vi "rename tag.vi"(7 "owner ID":string, 8 "error in":errorcluster, 9 "new name":string, 10 "old name":string, 11 "engine configuration in":refnum<class "engine configuration.lvclass">) -> (0 "error out":errorcluster, 3 "engine configuration out":refnum<class "engine configuration.lvclass">)   [LabVIEW 2014, in "engine configuration.lvclass"]
doc: "This function is used to rename a tag. If a tag claims to have an owner, only that owner is allowed to modify the tag name."
uses:
  engine configuration.lvclass
  <vilib>/NI/Tag Bus/tag/tag descriptor.lvclass
  <vilib>/NI/Tag Bus/tag/tag descriptor.lvclass/tag descriptor.ctl
  engine configuration.lvclass/engine configuration.ctl
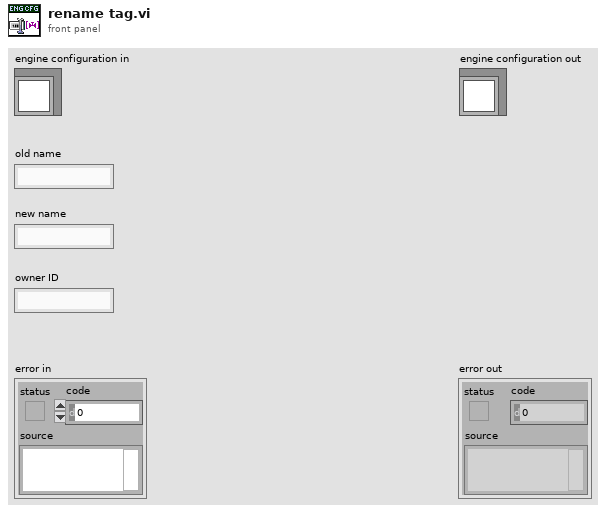
[diagram p1: front panel]
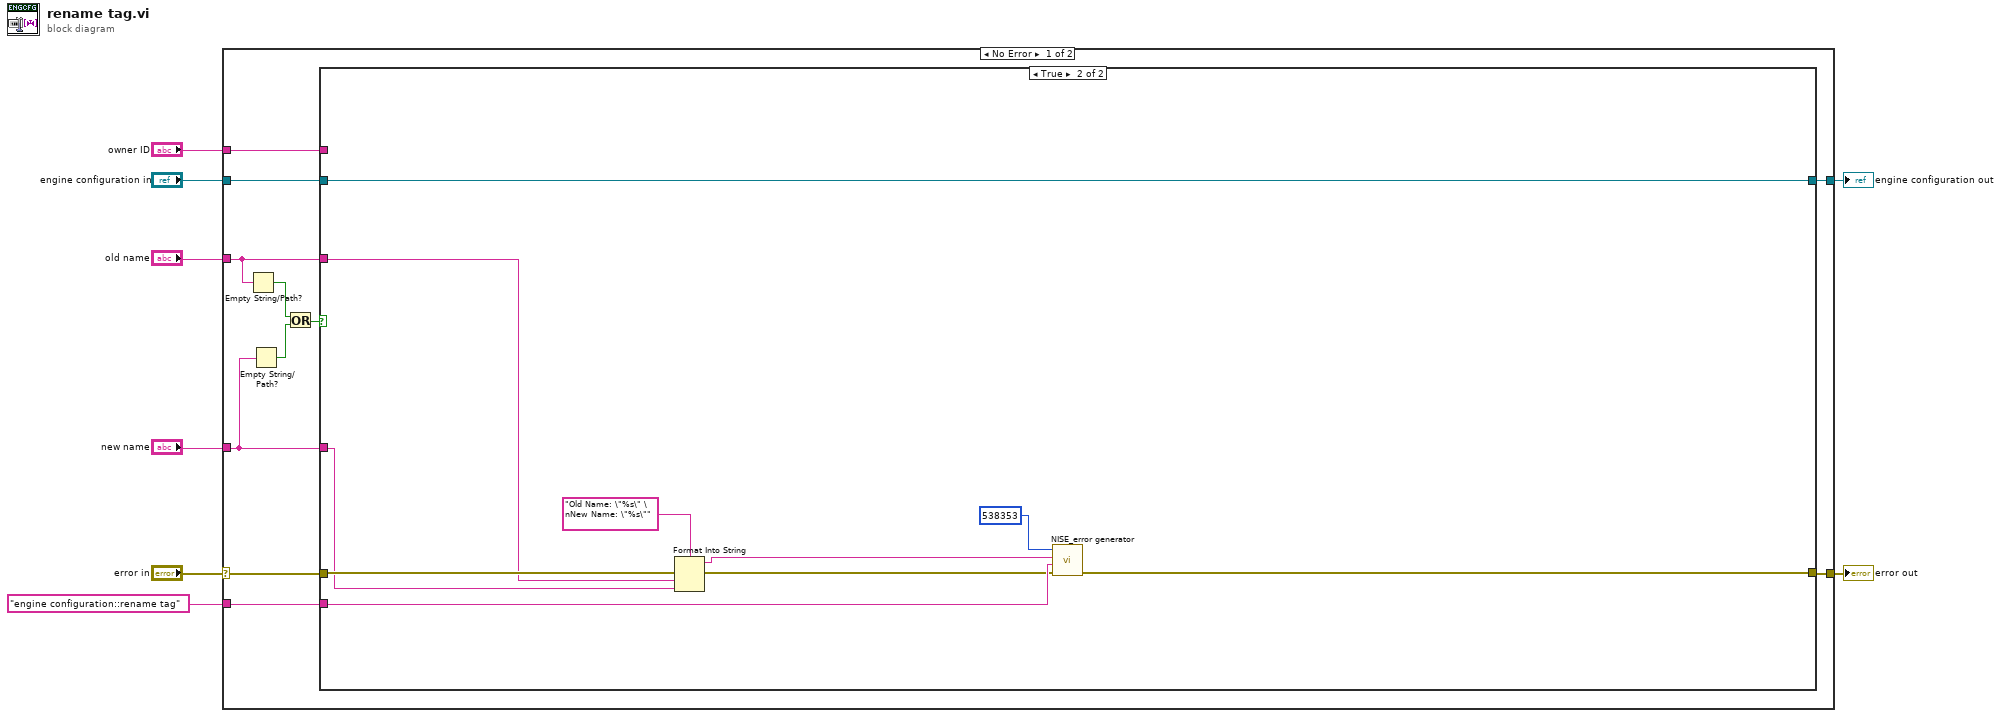
[diagram p0: block diagram]
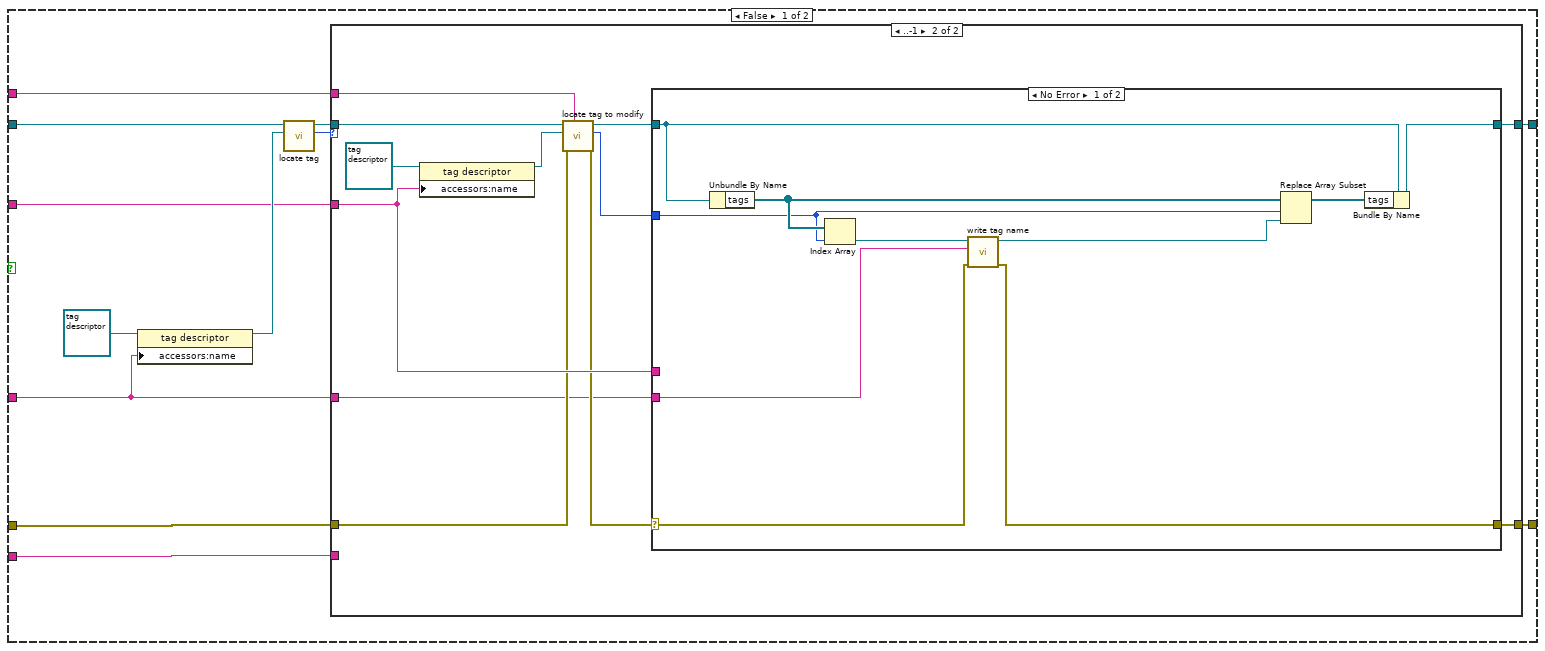
[diagram p2: hidden frame]
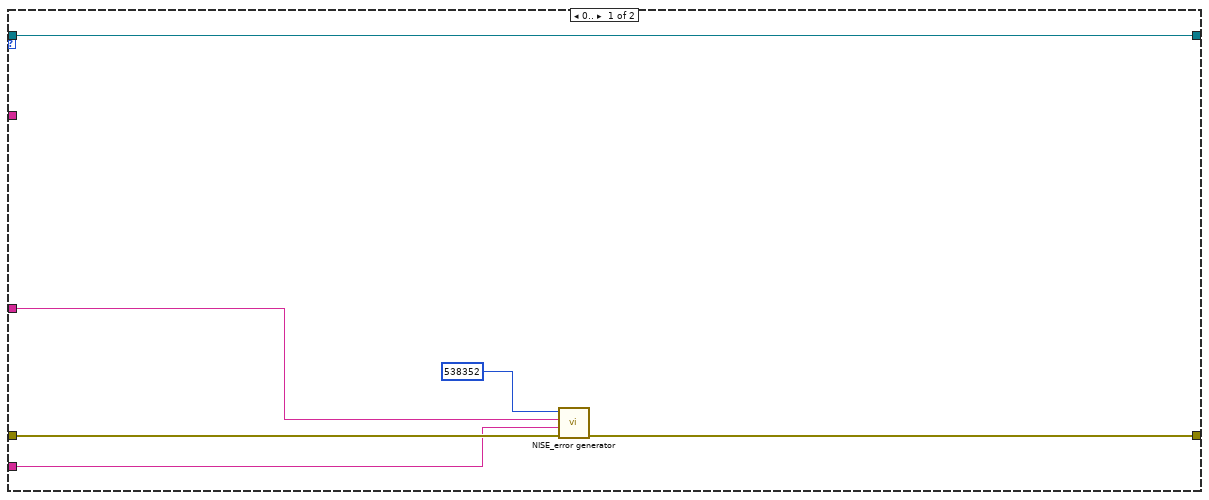
[diagram p3: hidden frame]
diagram:
  n1 = case shown="No Error" "error in" {
    selector: "error in" -> [w16 w73]
    tunnel: [w19 w73] -> w7
    tunnel: [w18 w72] -> w5
    tunnel: "engine configuration in" -> [w15 w72]
    tunnel: "old name" -> [w13 _]
    tunnel: "new name" -> [w12 _]
    tunnel: "owner ID" -> [w17 _]
    tunnel: "engine configuration::rename tag" ("source") -> [w14 _]
    frame No Error {
      n2 = Empty String/Path?(string/path=w13) -> (empty?=w10:bool)
      n3 = Empty String/Path?(string/path=w12) -> (empty?=w11:bool)
      n4 = Or(x=w10, y=w11) -> (x .or. y?=w9:bool)
      n5 = case shown="True" w9 {
        tunnel: [w31 w69] -> w19
        tunnel: [w30 w71] -> w18
        tunnel: w17 -> [w29 _]
        tunnel: w16 -> [w28 w70]
        tunnel: w15 -> [w27 w71]
        tunnel: w14 -> [w22 w68]
        tunnel: w13 -> [w21 w64]
        tunnel: w12 -> [w20 w63]
        frame False {
          n6 = property class="tag descriptor"(reference=refnum<class "tag descriptor.lvclass"> refnum ("tag descriptor"), "accessors:name"=w20) -> (reference out=w24:refnum<class "tag descriptor.lvclass">)  [unwired: 1 in, 1 out]
          n7 = call "locate tag.vi"("tag descriptor"=w24, "engine configuration in"=w27) -> ("index"=w23:i32, "engine configuration out"=w26:refnum<class "engine configuration.lvclass">)  [unwired: 8 in]
          n8 = case shown="..-1" w23 {
            tunnel: [w35 w48] -> w31
            tunnel: [w37 w47] -> w30
            tunnel: w21 -> [_ w46]
            tunnel: w29 -> [_ w44]
            tunnel: w28 -> [w36 w42]
            tunnel: w26 -> [w37 w39]
            tunnel: w20 -> [w34 w38]
            tunnel: w22 -> [w32 _]
            frame 0.. {
              n9 = call <vilib>:"NISE_error generator.vi"("error in"=w36, "source"=w32, "append error message"=w34, "error code (0)"=538352) -> ("error out"=w35:errorcluster)  [unwired: 5 in]
            }
            frame ..-1 {
              n10 = property class="tag descriptor"(reference=refnum<class "tag descriptor.lvclass"> refnum ("tag descriptor"), "accessors:name"=w46) -> (reference out=w43:refnum<class "tag descriptor.lvclass">)  [unwired: 1 in, 1 out]
              n11 = call "locate tag to modify.vi"("owner ID"=w44, "error in"=w42, "tag descriptor"=w43, "engine configuration in"=w39) -> ("error out"=w41:errorcluster, "index"=w40:i32, "engine configuration out"=w45:refnum<class "engine configuration.lvclass">)  [unwired: 5 in]
              n12 = case shown="No Error" w41 {
                selector: w41 -> [w52 w60]
                tunnel: [w51 w60] -> w48
                tunnel: w45 -> [w56 w61]
                tunnel: [w57 w61] -> w47
                tunnel: w38 -> [w50 _]
                tunnel: w46 -> [_ _]
                tunnel: w40 -> [w55 _]
                frame No Error {
                  n13 = Unbundle By Name(w56) -> ("tags"=w59:refnum<class "tag descriptor.lvclass">[])
                  n14 = Index Array(array=w59, index=w55) -> (element=w54:refnum<class "tag descriptor.lvclass">)
                  n15 = call <vilib>:"write tag name.vi"("error in"=w52, "name"=w50, "system tag in"=w54) -> ("error out"=w51:errorcluster, "system tag out"=w53:refnum<class "tag descriptor.lvclass">)  [unwired: 7 in]
                  n16 = Replace Array Subset(array=w59, new element=w53, index=w55) -> (w58:refnum<class "tag descriptor.lvclass">[])
                  n17 = Bundle By Name(cluster=w56, "tags"=w58) -> (w57:refnum<class "engine configuration.lvclass">)
                }
                frame Error {
                }
              }
            }
          }
        }
        frame True {
          n18 = Format Into String(format string="Old Name: \"%s\" \nNew Name: \"%s\"", error in=w70, w64, w63) -> (resulting string=w65:string, error out=w66:errorcluster)  [unwired: 1 in]
          n19 = call <vilib>:"NISE_error generator.vi"("error in"=w66, "source"=w68, "append error message"=w65, "error code (0)"=538353) -> ("error out"=w69:errorcluster)  [unwired: 5 in]
        }
      }
    }
    frame Error {
    }
  }
  "error out" <- w7
  "engine configuration out" <- w5
